vi "to string.vi"(8 "error in":errorcluster, 11 "Missing Plugin configuration in":refnum<class "Missing Plugin configuration.lvclass">) -> (0 "error out":errorcluster, 1 "data":string, 2 "version":string, 3 "Missing Plugin configuration out":refnum<class "Missing Plugin configuration.lvclass">)   [LabVIEW 2014, in "Missing Plugin configuration.lvclass"]
doc: "Provides an interface for saving a module configuration to a file or other serialized data source. It is recommended that all children of this class store data in two sets--data required for its own initialization, and any data required for parent initialization--and that each implementation uses the <b>Call Parent Method</b> primitive to serialize parent information."
uses:
  Missing Plugin configuration.lvclass
  current version.vi
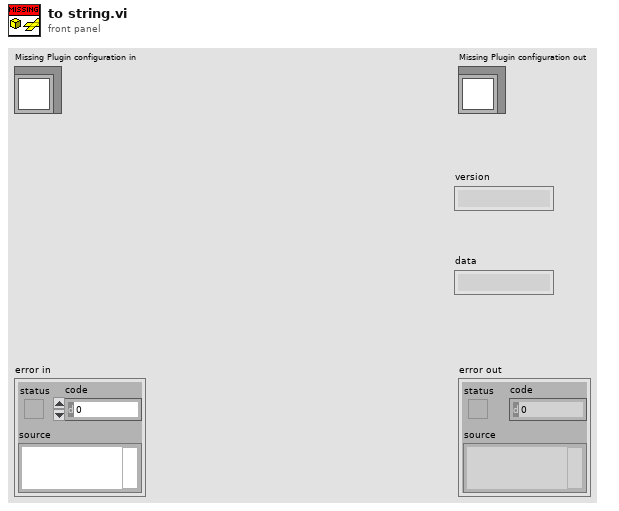
[diagram p1: front panel]
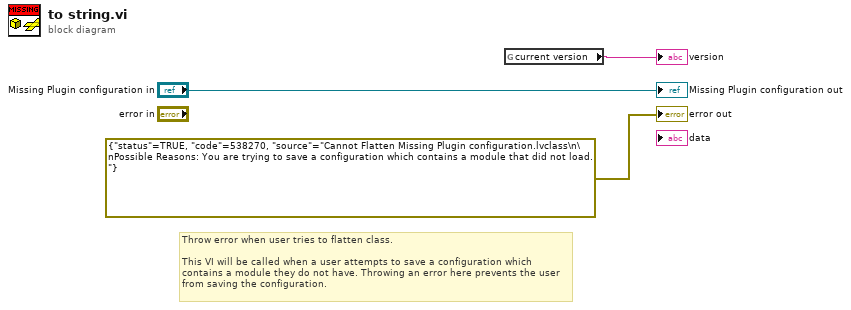
[diagram p0: block diagram]
diagram:
  # "Throw error when user tries to flatten class.\n\nThis VI will be called when a user attempts to save a configuration which contains a module they do not have. Throwing an error here prevents the user from saving the configuration."
  n1 = global read "current version.vi" "current version"() -> (→"version":string)
  "error out" <- errorcluster {"status"=TRUE, "code"=538270, "source"="Cannot Flatten Missing Plugin configuration.lvclass\n\nPossible Reasons: You are trying to save a configuration which contains a module that did not load."} ("error out")
  "Missing Plugin configuration out" <- "Missing Plugin configuration in"
